vi "Tempo_sec.vi"(1 "Temps sec":dbl) -> ()   [LabVIEW 2017]
panel:
  out "count ms":u32 caption="ms\nms"
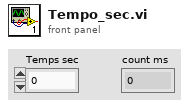
[diagram p1: front panel]
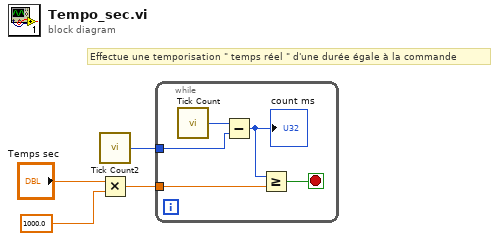
[diagram p0: block diagram]
diagram:
  # "Effectue une temporisation \" temps réel \" d'une durée égale à la commande"
  n1 = call "Tick Count2"() -> ("Tick Count(mSec)"=w4:u32)
  n2 = Multiply(x="Temps sec", y=1000.0) -> (x*y=w1:dbl)
  n3 = while {
    tunnel: w4 -> [w8]
    tunnel: w1 -> [w5]
    stop <- w6 stop-if-true
    n4 = call "Tick Count"() -> ("Tick Count(mSec)"=w9:u32)
    n5 = Subtract(x=w9, y=w8) -> (x-y=w7:u32)
    "count ms" <- w7
    n6 = Greater Or Equal?(x=w7, y=w5) -> (x >= y?=w6:bool)
  }
